vi "Add Fixture Custom URI.vi"(8 "error in (no error)":errorcluster, 11 "server id":i32) -> (0 "error out":errorcluster, 3 "server id out":i32)   [LabVIEW 2020, in "MCP Server tests.lvlib"]
doc: "Test helper. Registers the fixture file fixture_utf8.txt that lies beside this VI a second time as an MCP resource, under the custom uri test://fixture-text (the uri input of Add Resource (File).vi). Add Fixture Files.vi registers the same file under its derived uri labview://fixture_utf8."
uses:
  MCP Server tests.lvlib
  src/MCP Server/MCP Server.lvlib
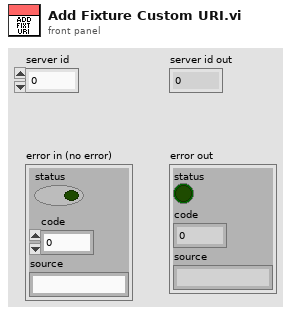
[diagram p1: front panel]
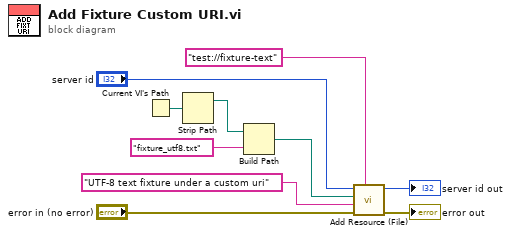
[diagram p0: block diagram]
diagram:
  n1 = Current VI's Path() -> (path=w8:path)
  n2 = Strip Path(path=w8) -> (stripped path=w9:path)  [unwired: 1 out]
  n3 = Build Path(base path=w9, name or relative path="fixture_utf8.txt" ("text fixture")) -> (appended path=w10:path)
  n4 = call "Add Resource (File).vi"("uri"="test://fixture-text", "error in (no error)"="error in (no error)", "description"="UTF-8 text fixture under a custom uri", "file path"=w10, "server id"="server id") -> ("error out"=→"error out":errorcluster, "server id out"=→"server id out":i32)  [unwired: 5 in]
